vi "Tidy Probe 3.vi"(0 "x":dbl) -> (4 "negative?":bool, 6 "joined":string, 8 "array":dbl[](array[numeric]))   [LabVIEW 2026]
doc: "Probe: constant labels, whitespace string, array constant, error constant, loop stop terminal, comparison with zero."
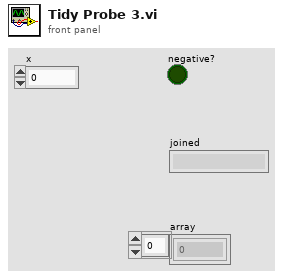
[diagram p1: front panel]
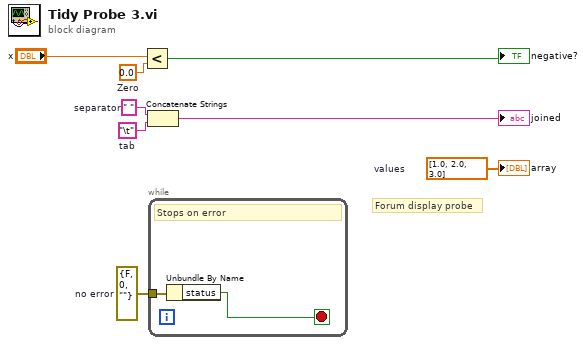
[diagram p0: block diagram]
diagram:
  w8 = errorcluster {"status"=FALSE, "code"=0, "source"=""}  # no error
  w7 = dbl[] [1.0, 2.0, 3.0]  # values
  w5 = "\t"  # tab
  w4 = " "  # separator
  w2 = 0.0  # Zero
  # "Forum display probe"
  n1 = Less?(x="x", y=w2) -> (x < y?=→"negative?":bool)
  n2 = Concatenate Strings(w4, w5) -> (→"joined":string)
  n3 = while {
    tunnel: w8 -> [w9]
    stop <- w10 stop-if-true
    # "Stops on error"
    n4 = Unbundle By Name(w9) -> ("status"=w10:bool)
  }
  "array" <- w7
